vi "Build Tool.vi"(6 "String":string, 7 "Ignored":string[](array[string])=["error in"], 8 "error in (no error)":errorcluster, 9 "Description":string, 11 "VI Refnum":refnum<vi>) -> (0 "error out":errorcluster, 3 "array":T1)   [LabVIEW 2020, in "MCP Server.lvlib"]
doc: "Creates a new Tool object from a VI."
uses:
  MCP Server.lvlib
  Output Parameter.ctl
  Input Parameter.ctl
  Tool Data.ctl
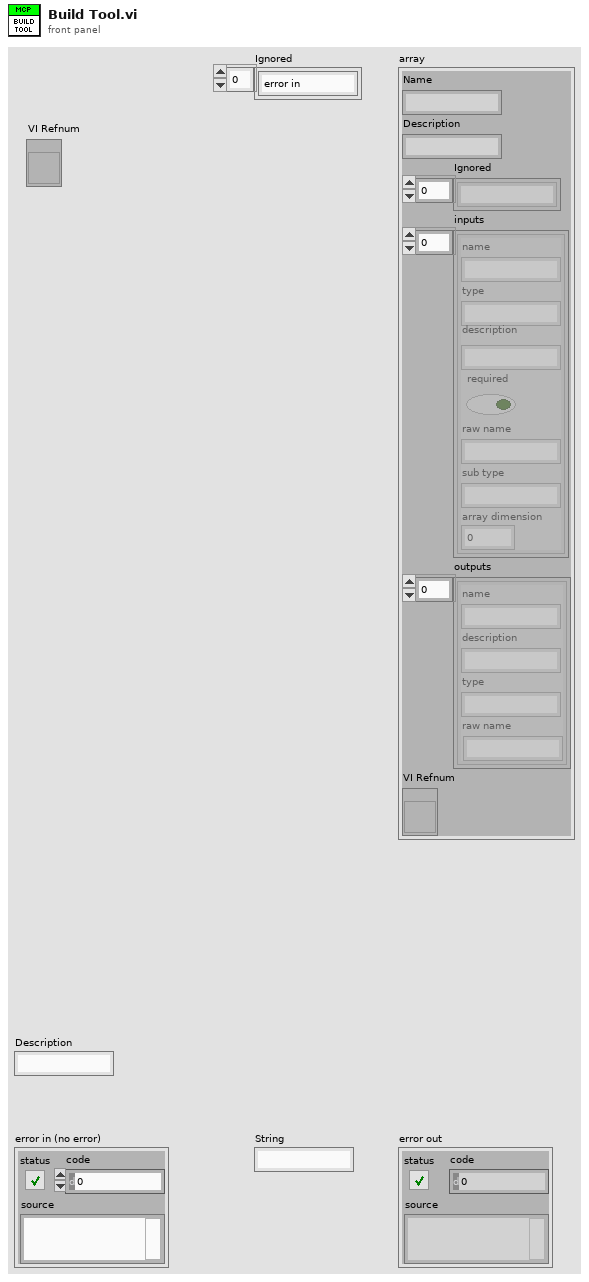
[diagram p1: front panel]
types:
  T1 = typedef "MCP Server.lvlib/Tool Data.ctl" = cluster{"Name":string, "Description":string, "Ignored":string[], "inputs":T2[], "outputs":T3[], "VI Refnum":refnum<vi>}
  T2 = typedef "MCP Server.lvlib/Input Parameter.ctl" = cluster{"name":string, "type":string, "description":string, "required":bool, "raw name":string, "sub type":string, "array dimension":i32}
  T3 = typedef "MCP Server.lvlib/Output Parameter.ctl" = cluster{"name":string, "description":string, "type":string, "raw name":string}
  T4 = typedef "MCP Server.lvlib/Terminal.ctl" = cluster{"Name":string, "Type":string, "IsIndicator?":bool, "IsRequired?":bool, "Description":string, "sub type":string, "array dimensions":i32}
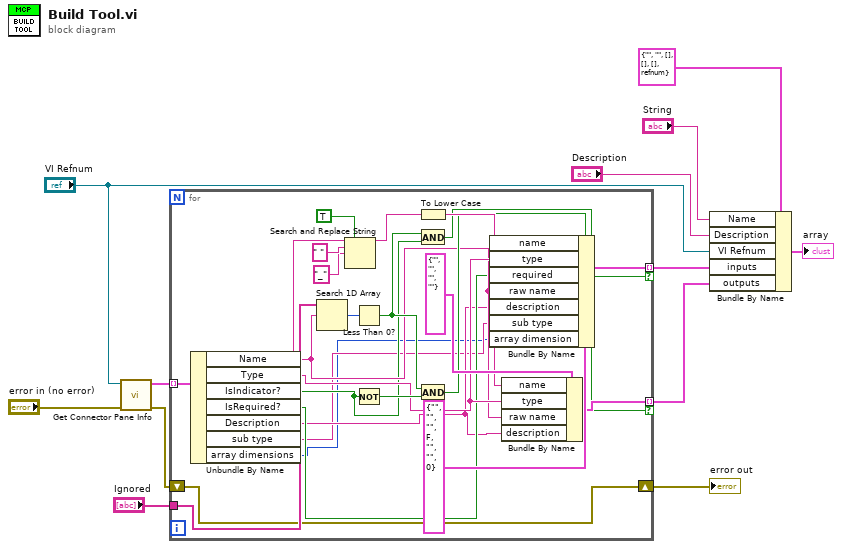
[diagram p0: block diagram]
diagram:
  n1 = call "Get Connector Pane Info.vi"("error in (no error)"="error in (no error)", "vi reference"="VI Refnum") -> ("error out"=w4:errorcluster, "Terminals"=w3:T4[])  [unwired: 8 in]
  n2 = for {
    tunnel: [w35] -> w9 mode=indexing if=w30
    tunnel: [w32] -> w10 mode=indexing if=w31
    tunnel: "Ignored" -> [w28]
    shift-right: [w25] -> w11
    shift-left: w4 -> [w25]
    tunnel: w3 -> [w20] mode=indexing
    n3 = Unbundle By Name(w20) -> ("Name"=w18:string, "Type"=w19:string, "IsIndicator?"=w16:bool, "IsRequired?"=w17:bool, "Description"=w15:string, "sub type"=w14:string, "array dimensions"=w13:i32)
    n4 = Search 1D Array(1D array=w28, element=w18) -> (index of element=w27:i32)  [unwired: 1 in]
    n5 = Search and Replace String(replace all?=TRUE ("replace all? (F)"), input string=w18, search string=" ", replace string="_" ("replace string (\"\")")) -> (result string=w24:string)  [unwired: 4 in, 3 out]
    n6 = Less Than 0?(x=w27) -> (x < 0?=w26:bool)
    n7 = Not(x=w16) -> (.not. x?=w29:bool)
    n8 = To Lower Case(string=w24) -> (all lower case string=w33:string)
    n9 = And(x=w26, y=w16) -> (x .and. y?=w31:bool)
    n10 = And(x=w26, y=w29) -> (x .and. y?=w30:bool)
    n11 = Bundle By Name(cluster=T2 {"name"="", "type"="", "description"="", "required"=FALSE, "raw name"="", "sub type"="", "array dimension"=0} ("Cluster"), "name"=w33, "type"=w19, "required"=w17, "raw name"=w18, "description"=w15, "sub type"=w14, "array dimension"=w13) -> (w35:T2)
    n12 = Bundle By Name(cluster=T3 {"name"="", "description"="", "type"="", "raw name"=""} ("outputs"), "name"=w33, "type"=w19, "raw name"=w18, "description"=w15) -> (w32:T3)
  }
  "error out" <- w11
  n13 = Bundle By Name(cluster=T1 {"Name"="", "Description"="", "Ignored"=[], "inputs"=[], "outputs"=[], "VI Refnum"=refnum} ("Tool Data"), "Name"="String", "Description"="Description", "VI Refnum"="VI Refnum", "inputs"=w9, "outputs"=w10) -> (→"array":T1)
